vi "ParseVectorFile.SVG.ImageFactory.vi"(8 "error in (no error)":errorcluster, 11 "ParseVectorFile in":refnum<class "ParseVectorFile.lvclass">) -> (0 "error out":errorcluster, 3 "ParseVectorFile out":refnum<class "ParseVectorFile.lvclass">)   [LabVIEW 2019, in "ParseVectorFile.lvclass"]
uses:
  ParseVectorFile.lvclass
  ParseVectorFile.lvclass/ParseVectorFile.ctl
  ParseXML/ParseSVG.lvclass/ParseSVG.ctl
  Image/SVGImage.lvclass
  Image/InitializationInfo.ctl
  ParseXML/Image.ctl
  ParseXML/ParseSVG.lvclass
  EditSVG/EditSVG.lvclass
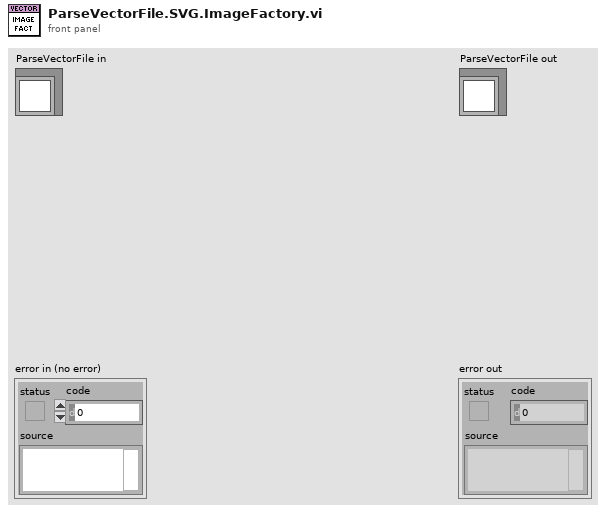
[diagram p1: front panel]
types:
  T1 = typedef "ParseSVG.lvclass/Image.ctl" = cluster{"x":string, "y":string, "width":string, "height":string, "xlink:href":string, "id":string, "transform":string}
  T2 = enum16{"open", "replace", "create", "open or create", "replace or create", "replace or create with confirmation"}
  T3 = typedef "SVGImage.lvclass/InitializationInfo.ctl" = cluster{"X":string, "Y":string, "Width":string, "Height":string, "File Path":string, "ID":string, "transform":string}
  T4 = cluster{"Backmost?":bool, "Correct location?":bool, "Surface Pic?":bool, "Correct Name?":bool}
  T5 = cluster{"Node Name":string, "Node SVG ID":string, "Attribute Name":string, "New Attribute Value":string}
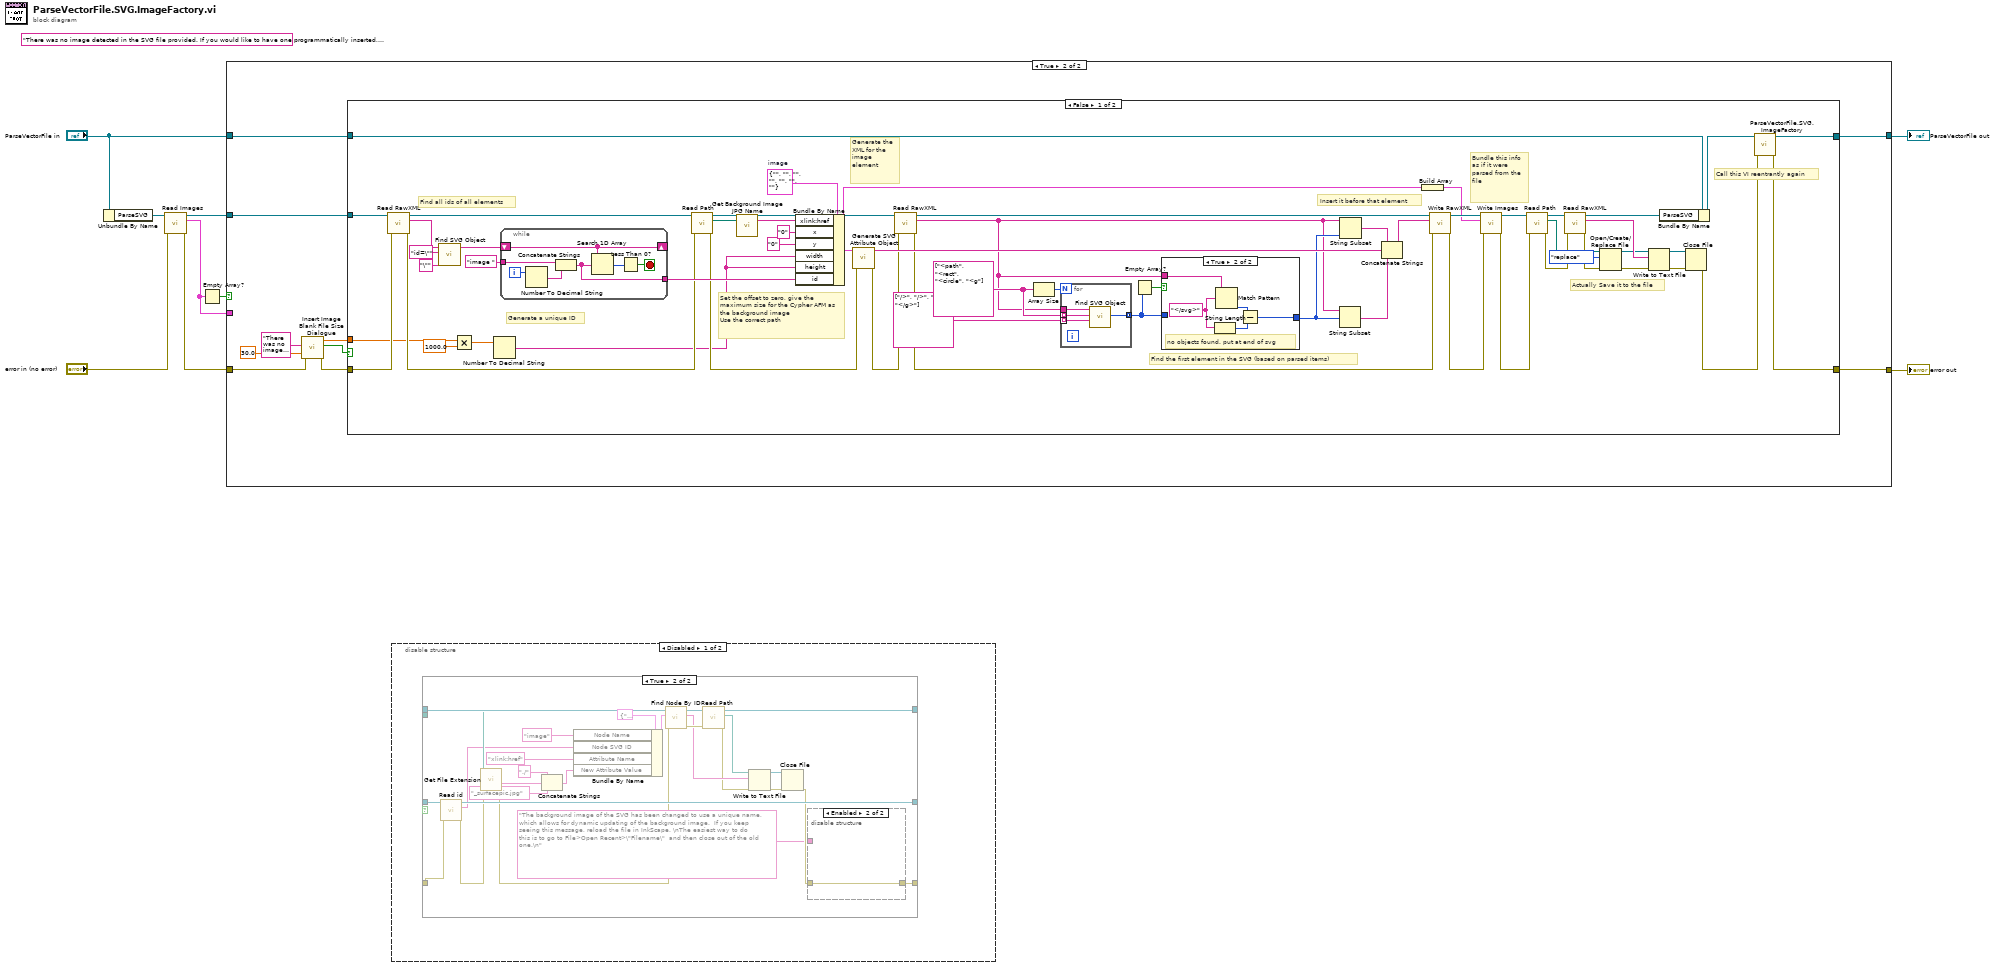
[diagram p0: block diagram]
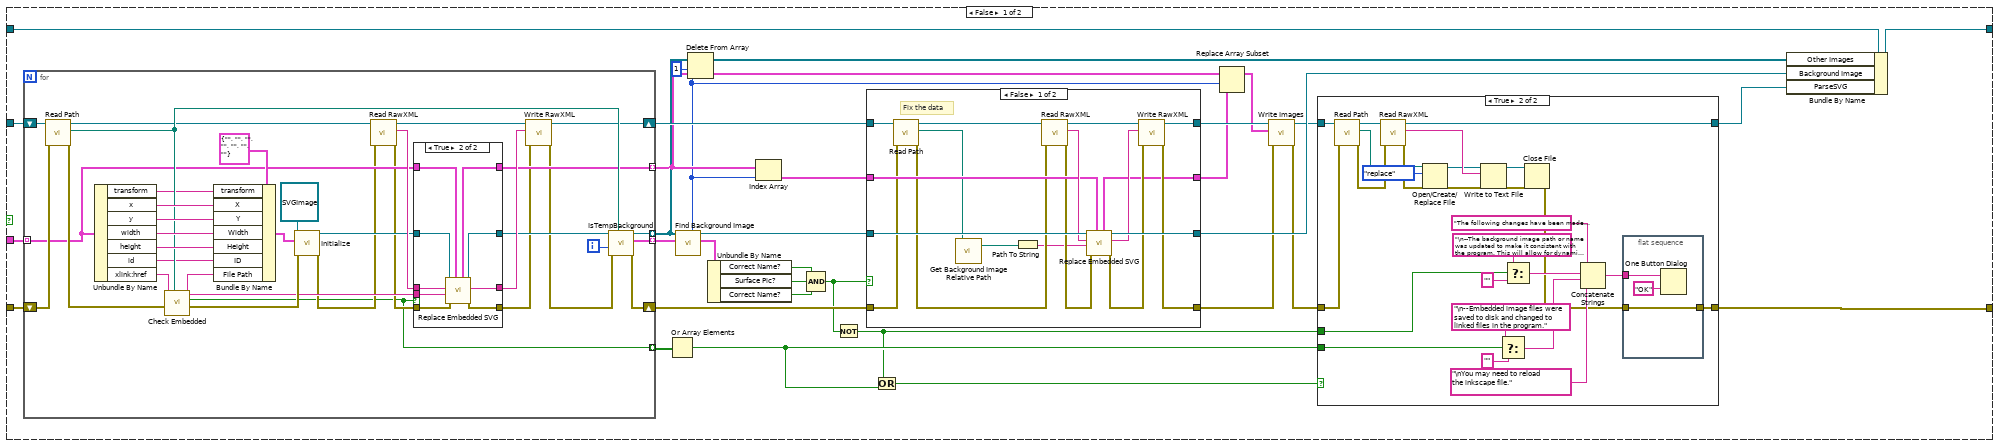
[diagram p2: hidden frame]
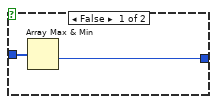
[diagram p6: hidden frame]
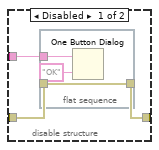
[diagram p9: hidden frame]
diagram:
  (unwired) "There was no image detected in the SVG file provided. If you would like to have one programmatically inserted, please input the correct image size below in um, and press OK. If you would prefer to do this yourself, press Cancel." ("Message to User")
  n1 = Unbundle By Name("ParseVectorFile in") -> ("ParseSVG"=w7:refnum<class "ParseSVG.lvclass">)
  n2 = call "Read Images.vi"("error in (no error)"="error in (no error)", "ParseSVG in"=w7) -> ("error out"=w3:errorcluster, "Images"=w1:T1[], "ParseSVG out"=w4:refnum<class "ParseSVG.lvclass">)  [unwired: 7 in]
  n3 = Empty Array?(array=w1) -> (empty?=w2:bool)
  n4 = case shown="True" w2 {
    tunnel: [w42 w151] -> w8
    tunnel: "ParseVectorFile in" -> [w41 w144]
    tunnel: [w40 w143] -> w5
    tunnel: w4 -> [w24 w152]
    tunnel: w1 -> [w23 _]
    tunnel: w3 -> [w22 w147]
    frame False {
      n5 = for {
        shift-right: [w124] -> w28
        shift-left: w22 -> [w116]
        tunnel: w23 -> [w105] mode=indexing
        shift-right: [w111] -> w29
        shift-left: w24 -> [w117]
        tunnel: [w125] -> w20 mode=indexing
        tunnel: [w120] -> w36 mode=indexing
        tunnel: [w102] -> w15 mode=indexing
        tunnel: [w97] -> w27 mode=indexing
        i -> [w119]
        n6 = call-dynamic "Read Path.vi"("error in (no error)"=w116, "ParseSVG in"=w117) -> ("error out"=w115:errorcluster, "Path"=w113:path, "ParseSVG out"=w112:refnum<class "ParseSVG.lvclass">)  [unwired: 7 in]
        n7 = Unbundle By Name(w105) -> ("transform"=w96:string, "x"=w129:string, "y"=w128:string, "width"=w127:string, "height"=w126:string, "id"=w110:string, "xlink:href"=w114:string)
        n8 = call "Check Embedded.vi"("SVG Path"=w113, "error in (no error)"=w115, "URI"=w114) -> ("error out"=w118:errorcluster, "Embedded"=w97:bool, "Path Out"=w106:string)  [unwired: 6 in]
        n9 = Bundle By Name(cluster=T3 {"X"="", "Y"="", "Width"="", "Height"="", "File Path"="", "ID"="", "transform"=""} ("Info"), "transform"=w96, "X"=w129, "Y"=w128, "Width"=w127, "Height"=w126, "ID"=w110, "File Path"=w106) -> (w122:T3)
        n10 = call "Initialize.vi"("error in (no error)"=w118, "Info"=w122, "Image in"=refnum<class "SVGImage.lvclass"> refnum) -> ("error out"=w101:errorcluster, "Image out"=w104:refnum<class "SVGImage.lvclass">)  [unwired: 7 in]
        n11 = call "Read RawXML.vi"("error in (no error)"=w101, "ParseXML in"=w112) -> ("error out"=w100:errorcluster, "RawXML"=w108:string, "ParseXML out"=w109:refnum<class "ParseSVG.lvclass">)  [unwired: 7 in]
        n12 = case shown="True" w97 {
          tunnel: [w132 w142] -> w99
          tunnel: w100 -> [w132 w141]
          tunnel: w108 -> [w131 w140]
          tunnel: [w131 w139] -> w107
          tunnel: w106 -> [_ w138]
          tunnel: w105 -> [w130 w134]
          tunnel: w104 -> [w133 w137]
          tunnel: [w133 w136] -> w103
          tunnel: [w130 w135] -> w102
          frame False {
          }
          frame True {
            n13 = call "Replace Embedded SVG.vi"("image"=w134, "error in"=w141, "xlink:href"=w138, "XML In"=w140, "SVGImage in"=w137) -> ("error out"=w142:errorcluster, "Edited XML Out"=w139:string, "SVGImage out"=w136:refnum<class "SVGImage.lvclass">, "image out"=w135:T1)  [unwired: 3 in]
          }
        }
        n14 = call "Write RawXML.vi"("error in (no error)"=w99, "RawXML"=w107, "ParseSVG.lvclass"=w109) -> ("error out"=w98:errorcluster, "ParseSVG.lvclass 2"=w111:refnum<class "ParseSVG.lvclass">)  [unwired: 7 in]
        n15 = call "IsTempBackground.vi"("SVG Path"=w113, "error in"=w98, "Order (back to front)"=w119, "SVGImage in"=w103) -> ("error out"=w124:errorcluster, "Backgroundic Qualities"=w120:T4, "SVGImage out"=w125:refnum<class "SVGImage.lvclass">)  [unwired: 5 in]
      }
      n16 = Or Array Elements(Boolean array=w27) -> (logical OR=w19:bool)
      n17 = call "Find Background Image.vi"("Backgroundic Qualities"=w36, "Images"=w20) -> ("Backgroundic Qualities"=w34:T4, "Background Image"=w35:refnum<class "SVGImage.lvclass">, "Index"=w14:i32)  [unwired: 7 in]
      n18 = Delete From Array(array=w20, length=1, index=w14) -> (array with subset deleted=w37:refnum<class "SVGImage.lvclass">[])  [unwired: 1 out]
      n19 = Unbundle By Name(w34) -> ("Correct Name?"=w31:bool, "Surface Pic?"=w33:bool, "Correct Name?"=w32:bool)
      n20 = Index Array(array=w15, index=w14) -> (element=w30:T1)
      n21 = Compound Arithmetic op=AND(w31, w33, w32) -> (w26:bool)
      n22 = Not(x=w26) -> (.not. x?=w18:bool)
      n23 = case shown="False" w26 {
        tunnel: w35 -> [w88 w94]
        tunnel: [w90 w95] -> w17
        tunnel: w29 -> [w91 w95]
        tunnel: [w89 w94] -> w39
        tunnel: w30 -> [w83 w92]
        tunnel: w28 -> [w79 w93]
        tunnel: [w80 w93] -> w11
        tunnel: [w74 w92] -> w13
        frame False {
          # "Fix the data"
          n24 = call-dynamic "Read Path.vi"("error in (no error)"=w79, "ParseSVG in"=w91) -> ("error out"=w78:errorcluster, "Path"=w77:path, "ParseSVG out"=w87:refnum<class "ParseSVG.lvclass">)  [unwired: 7 in]
          n25 = call "Get Background Image Relative Path.vi"("Inkscape Path"=w77) -> ("Relative Path to Background"=w76:path)  [unwired: 2 in]
          n26 = Path To String(path=w76) -> (string=w75:string)
          n27 = call "Read RawXML.vi"("error in (no error)"=w78, "ParseXML in"=w87) -> ("error out"=w82:errorcluster, "RawXML"=w85:string, "ParseXML out"=w86:refnum<class "ParseSVG.lvclass">)  [unwired: 7 in]
          n28 = call "Replace Embedded SVG.vi"("image"=w83, "error in"=w82, "xlink:href"=w75, "XML In"=w85, "SVGImage in"=w88) -> ("error out"=w81:errorcluster, "Edited XML Out"=w84:string, "SVGImage out"=w89:refnum<class "SVGImage.lvclass">, "image out"=w74:T1)  [unwired: 3 in]
          n29 = call "Write RawXML.vi"("error in (no error)"=w81, "RawXML"=w84, "ParseSVG.lvclass"=w86) -> ("error out"=w80:errorcluster, "ParseSVG.lvclass 2"=w90:refnum<class "ParseSVG.lvclass">)  [unwired: 7 in]
        }
        frame True {
        }
      }
      n30 = Or(x=w18, y=w19) -> (x .or. y?=w25:bool)
      n31 = Replace Array Subset(array=w15, new element=w13, index=w14) -> (w12:T1[])
      n32 = call "Write Images.vi"("error in (no error)"=w11, "Images"=w12, "ParseSVG in"=w17) -> ("error out"=w10:errorcluster, "ParseSVG out"=w16:refnum<class "ParseSVG.lvclass">)  [unwired: 7 in]
      n33 = case shown="True" w25 {
        tunnel: w16 -> [w43 w68]
        tunnel: w10 -> [w44 w64]
        tunnel: [w44 w46] -> w42
        tunnel: [w43 w63] -> w38
        tunnel: w18 -> [_ w56]
        tunnel: w19 -> [_ w55]
        frame False {
        }
        frame True {
          n34 = call-dynamic "Read Path.vi"("error in (no error)"=w64, "ParseSVG in"=w68) -> ("error out"=w58:errorcluster, "Path"=w66:path, "ParseSVG out"=w67:refnum<class "ParseSVG.lvclass">)  [unwired: 7 in]
          n35 = call "Read RawXML.vi"("error in (no error)"=w58, "ParseXML in"=w67) -> ("error out"=w59:errorcluster, "RawXML"=w70:string, "ParseXML out"=w63:refnum<class "ParseSVG.lvclass">)  [unwired: 7 in]
          n36 = Open/Create/Replace File(file path (use dialog)=w66, error in=w59, operation (0:open)=T2."replace") -> (refnum out=w69:refnum<file>, error out=w61:errorcluster)  [unwired: 3 in, 1 out]
          n37 = Write to Text File(file (use dialog)=w69, text=w70, error in=w61) -> (refnum out=w65:refnum<file>, error out=w60:errorcluster)  [unwired: 1 in, 1 out]
          n38 = Select(t="\n--Embedded image files were saved to disk and changed to linked files in the program.", s=w55, f="") -> (s? t:f=w50:string)
          n39 = Select(t="\n--The background image path or name was updated to make it consistent with the program. This will allow for dynamic updating if the AFM image, page, or data range is changed.", s=w56, f="") -> (s? t:f=w51:string)
          n40 = Close File(refnum=w65, error in=w60) -> (error out=w47:errorcluster)  [unwired: 1 out]
          n41 = Concatenate Strings("The following changes have been made to the inkscape file:", w51, w50, "\nYou may need to reload the inkscape file." ("string")) -> (w48:string)
          n42 = flat-sequence {
            tunnel: w48 -> [w72]
            tunnel: w47 -> [w71]
            tunnel: [w71] -> w46
            frame #0 {
              n43 = One Button Dialog(message=w72, button name ("OK")="OK") -> ()  [unwired: 1 out]
            }
          }
        }
      }
      n44 = Bundle By Name(cluster=w41, "Other Images"=w37, "Background Image"=w39, "ParseSVG"=w38) -> (w40:refnum<class "ParseVectorFile.lvclass">)
    }
    frame True {
      n45 = call "Insert Image Blank File Size Dialogue.vi"("Error In"=w147, "Message to User"="There was no image detected in the SVG file provided. If you would like to have one programmatically inserted, please input the correct image size below in um, and press OK. If you would prefer to do this yourself, press Cancel.", "Scan Size (um)"=30.0) -> ("Error Out"=w148:errorcluster, "Cancelled?"=w145:bool, "Scan Size Out"=w146:dbl)  [unwired: 6 in]
      n46 = case shown="False" w145 {
        tunnel: w152 -> [w190 _]
        tunnel: w148 -> [w185 w229]
        tunnel: [w160 w229] -> w151
        tunnel: w146 -> [w175 _]
        tunnel: w144 -> [w165 w228]
        tunnel: [w162 w228] -> w143
        frame False {
          w197 = string[] ["<path", "<rect", "<circle", "<g"]
          w208 = T1 {"x"="", "y"="", "width"="", "height"="", "xlink:href"="", "id"="", "transform"=""}  # image
          # "Call this VI reentrantly again"
          # "Actually Save it to the file"
          # "Bundle this info as if it were parsed from the file"
          # "Generate the XML for the image element"
          # "Find all ids of all elements"
          # "Insert it before that element"
          # "Find the first element in the SVG (based on parsed items)"
          # "Generate a unique ID"
          # "Set the offset to zero, give the maximum size for the Cypher AFM as the background image\nUse the correct path"
          n47 = call "Read RawXML.vi"("error in (no error)"=w185, "ParseXML in"=w190) -> ("error out"=w189:errorcluster, "RawXML"=w200:string, "ParseXML out"=w209:refnum<class "ParseSVG.lvclass">)  [unwired: 7 in]
          n48 = call "Find SVG Object.vi"("Ending Delimiter"="\"", "Beginning Delimiter"="id=\"", "XML String"=w200) -> ("Found Values"=w203:string[])  [unwired: 6 in, 2 out]
          n49 = Multiply(x=w175, y=1000.0) -> (x*y=w173:dbl)
          n50 = Number To Decimal String(number=w173) -> (decimal integer string=w172:string)  [unwired: 1 in]
          n51 = while {
            shift-right: [w224] -> _
            shift-left: w203 -> [w224]
            tunnel: "image " -> [w226]
            tunnel: [w223] -> w201
            i -> [w227]
            stop <- w222 stop-if-true
            n52 = Number To Decimal String(number=w227) -> (decimal integer string=w221:string)  [unwired: 1 in]
            n53 = Concatenate Strings(w226, w221) -> (w223:string)
            n54 = Search 1D Array(1D array=w224, element=w223) -> (index of element=w225:i32)  [unwired: 1 in]
            n55 = Less Than 0?(x=w225) -> (x < 0?=w222:bool)
          }
          n56 = call-dynamic "Read Path.vi"("error in (no error)"=w189, "ParseSVG in"=w209) -> ("error out"=w186:errorcluster, "Path"=w159:path, "ParseSVG out"=w196:refnum<class "ParseSVG.lvclass">)  [unwired: 7 in]
          n57 = call "Get Background Image JPG Name.vi"("Inkscape Path"=w159) -> ("Background JPG Name"=w158:string)  [unwired: 2 in]
          n58 = Bundle By Name(cluster=w208, "xlink:href"=w158, "x"="0", "y"="0", "width"=w172, "height"=w172, "id"=w201) -> (w171:T1)
          n59 = call "Generate SVG Attribute Object.vi"("error in (no error)"=w186, "Named Cluster of Data"=w171) -> ("error out"=w187:errorcluster, "SVG Attribute Object"=w193:string)  [unwired: 8 in]
          n60 = call "Read RawXML.vi"("error in (no error)"=w187, "ParseXML in"=w196) -> ("error out"=w188:errorcluster, "RawXML"=w154:string, "ParseXML out"=w192:refnum<class "ParseSVG.lvclass">)  [unwired: 7 in]
          n61 = Array Size(array=w197) -> (size(s)=w199:i32)
          n62 = for {
            N: w199 -> [_]
            tunnel: w154 -> [w220]
            tunnel: w197 -> [w219] mode=indexing
            tunnel: string[] ["/>", "/>", "/>", "</g>"] -> [w218] mode=indexing
            tunnel: [w217] -> w156 mode=concatenating
            n63 = call "Find SVG Object.vi"("Ending Delimiter"=w218, "Beginning Delimiter"=w219, "XML String"=w220) -> ("Beginning Indices"=w217:i32[])  [unwired: 6 in, 2 out]
          }
          n64 = Empty Array?(array=w156) -> (empty?=w157:bool)
          n65 = case shown="True" w157 {
            tunnel: w156 -> [w211 _]
            tunnel: [w210 w214] -> w155
            tunnel: w154 -> [_ w213]
            frame False {
              n66 = Array Max & Min(array=w211) -> (min value=w210:i32)  [unwired: 3 out]
            }
            frame True {
              w212 = "</svg>" ("regular expression")
              # "no objects found. put at end of svg"
              n67 = String Length(string=w212) -> (length=w216:i32)
              n68 = Match Pattern(string=w213, regular expression=w212) -> (offset past match=w215:i32)  [unwired: 1 in, 3 out]
              n69 = Subtract(x=w215, y=w216) -> (x-y=w214:i32)
            }
          }
          n70 = String Subset(string=w154, offset (0)=w155) -> (substring=w194:string)  [unwired: 1 in]
          n71 = String Subset(string=w154, length (rest)=w155) -> (substring=w195:string)  [unwired: 1 in]
          n72 = Concatenate Strings(w195, w193, w194) -> (w191:string)
          n73 = Build Array(w171) -> (w168:T1[])
          n74 = call "Write RawXML.vi"("error in (no error)"=w188, "RawXML"=w191, "ParseSVG.lvclass"=w192) -> ("error out"=w167:errorcluster, "ParseSVG.lvclass 2"=w170:refnum<class "ParseSVG.lvclass">)  [unwired: 7 in]
          n75 = call "Write Images.vi"("error in (no error)"=w167, "Images"=w168, "ParseSVG in"=w170) -> ("error out"=w166:errorcluster, "ParseSVG out"=w169:refnum<class "ParseSVG.lvclass">)  [unwired: 7 in]
          n76 = call-dynamic "Read Path.vi"("error in (no error)"=w166, "ParseSVG in"=w169) -> ("error out"=w176:errorcluster, "Path"=w181:path, "ParseSVG out"=w182:refnum<class "ParseSVG.lvclass">)  [unwired: 7 in]
          n77 = call "Read RawXML.vi"("error in (no error)"=w176, "ParseXML in"=w182) -> ("error out"=w177:errorcluster, "RawXML"=w184:string, "ParseXML out"=w164:refnum<class "ParseSVG.lvclass">)  [unwired: 7 in]
          n78 = Open/Create/Replace File(file path (use dialog)=w181, error in=w177, operation (0:open)=T2."replace") -> (refnum out=w183:refnum<file>, error out=w179:errorcluster)  [unwired: 3 in, 1 out]
          n79 = Write to Text File(file (use dialog)=w183, text=w184, error in=w179) -> (refnum out=w180:refnum<file>, error out=w178:errorcluster)  [unwired: 1 in, 1 out]
          n80 = Bundle By Name(cluster=w165, "ParseSVG"=w164) -> (w163:refnum<class "ParseVectorFile.lvclass">)
          n81 = Close File(refnum=w180, error in=w178) -> (error out=w161:errorcluster)  [unwired: 1 out]
          n82 = call "ParseVectorFile.SVG.ImageFactory.vi"("error in (no error)"=w161, "ParseVectorFile in"=w163) -> ("error out"=w160:errorcluster, "ParseVectorFile out"=w162:refnum<class "ParseVectorFile.lvclass">)  [unwired: 8 in]
        }
        frame True {
          # "User wants to just move on..."
        }
      }
    }
  }
  "error out" <- w8
  "ParseVectorFile out" <- w5
  n83 = disable-structure shown="Disabled" {
    frame Disabled {
      n84 = case shown="True" {
        selector: _ -> [_ _]
        tunnel: _ -> [w232 w259]
        tunnel: [w232 w251] -> _
        tunnel: [w230 w234] -> _
        tunnel: _ -> [w231 w258]
        tunnel: _ -> [w230 w257]
        tunnel: [w231 w256] -> _
        tunnel: _ -> [_ w242]
        frame False {
        }
        frame True {
          n85 = call-dynamic "Read id.vi"("error in (no error)"=w257, "SVG Object in"=w258) -> ("error out"=w244:errorcluster, "id"=w239:string, "SVG Object out"=w256:refnum<class "SVGImage.lvclass">)  [unwired: 7 in]
          n86 = call <vilib>:"Get File Extension.vi"("error in (no error)"=w244, "file"=w242) -> ("error out"=w243:errorcluster, "filename without extension"=w237:string)  [unwired: 5 in, 3 out]
          n87 = Concatenate Strings("./" ("string"), w237, "_surfacepic.jpg" ("string")) -> (w240:string)
          n88 = Bundle By Name(cluster=T5 {"Node Name"="", "Node SVG ID"="", "Attribute Name"="", "New Attribute Value"=""} ("Node Info"), "Node Name"="image" ("Node Name (exact)"), "Node SVG ID"=w239, "Attribute Name"="xlink:href", "New Attribute Value"=w240) -> (w253:T5)
          n89 = call "Find Node By ID.vi"("error in (no error)"=w243, "Node Info"=w253, "ParseSVG in"=w259) -> ("error out"=w250:errorcluster, "Corrected XML"=w249:string, "ParseSVG out"=w252:refnum<class "ParseSVG.lvclass">)  [unwired: 6 in]
          n90 = call-dynamic "Read Path.vi"("error in (no error)"=w250, "ParseSVG in"=w252) -> ("error out"=w247:errorcluster, "Path"=w248:path, "ParseSVG out"=w251:refnum<class "ParseSVG.lvclass">)  [unwired: 7 in]
          n91 = Write to Text File(file (use dialog)=w248, text=w249, error in=w247) -> (refnum out=w246:refnum<file>, error out=w245:errorcluster)  [unwired: 1 in, 1 out]
          n92 = Close File(refnum=w246, error in=w245) -> (error out=w235:errorcluster)  [unwired: 1 out]
          n93 = disable-structure shown="Enabled" {
            disable-tunnel: w235 -> [w262 w266]
            disable-tunnel: [w261 w266] -> w234
            disable-tunnel: "The background image of the SVG has been changed to use a unique name, which allows for dynamic updating of the background image.  If you keep seeing this message, reload the file in InkScape. \nThe easiest way to do this is to go to File>Open Recent>\"Filename\"  and then close out of the old one.\n" ("message") -> [w260 _]
            frame Disabled {
              n94 = flat-sequence {
                tunnel: w262 -> [w265]
                tunnel: [w265] -> w261
                tunnel: w260 -> [w264]
                frame #0 {
                  n95 = One Button Dialog(message=w264, button name ("OK")="OK") -> ()  [unwired: 1 out]
                }
              }
            }
            frame Enabled {
            }
          }
        }
      }
    }
    frame Enabled {
    }
  }
